vi "AT1B_Naeherung.vi"() -> ()   [LabVIEW 2026]
doc: "Virtueller Schlitten. NJ8 verwendet typische Daten, CJ8 und seitliche Geometrie sind einstellbare Beispiele. Erst Sensor und Probe waehlen, dann axial oder seitlich\nfahren. Nullsetzen aendert nur den Massstab."
panel:
  out "Bewegungsparameter gueltig":bool=TRUE
  out "Grafikfehlercode":i32
  out "Ausgangsspannung [V] - 20 ms je Punkt":dbl(graph)
  out "CSV-Fehlercode":i32
  out "Ungespeicherte Daten":bool
  out "Zeilen aufgenommen":i32
  out "Aufnahmestatus":string
  in  "Pruefstand beenden":bool
  in  "Neue CSV-Datei":path
  in  "CSV speichern":bool
  in  "Ungespeicherte Aufnahme verwerfen erlauben":bool
  in  "Neue Aufnahme":bool
  in  "Aufnahme eingeschaltet":bool
  out "Signalzustand":string="Mit Ausfuehren / Strg+R starten."
  out "Messung angehalten - Anzeige historisch":bool
  out "Massstab x [mm]":dbl=nan
  out "Massstab s [mm]":dbl=nan
  out "Ausgangsspannung [V]":dbl=nan
  out "Schaltausgang":bool
  in  "Messung eingeschaltet":bool=TRUE
  in  "Materialfaktor (-1 = Vorbelegung)":dbl=-1.0
  in  "Massstab x nullen":bool
  in  "Massstab s nullen":bool
  in  "Seitliche Reichweite [mm] - Beispiel":dbl=12.0
  in  "Hysterese-Anteil - Beispiel":dbl=0.075
  in  "CJ8 Empfindlichkeit [0..1]":dbl=0.5
  in  "Sensor eingeschaltet":bool=TRUE
  in  "Probenbreite [mm] (24 oder 40)":dbl=24.0
  in  "Andere Achse [mm]":dbl
  in  "Bewegte Achse":enum16{"Axial s", "Seitlich x"}(ring)
  in  "Probe (NJ8 / CJ8 Reihenfolge)":T1(ring)
  in  "Sensor":enum16{"NJ8 induktiv", "CJ8 kapazitiv"}(ring)
  out "Abgeschlossene Fahrten":dbl
  out "Fahrt aktiv":bool
  out "Position aktuell":dbl
  in  "Bewegung pausieren":bool
  in  "Bewegung stoppen":bool
  in  "Ablauf starten":bool
  in  "Schrittweite":dbl=0.1
  in  "Fahrtart":enum16{"Pendeln", "Schritte", "Einfachfahrt"}(ring)
  in  "Wiederholungen":dbl=1.0
  in  "Haltezeit [s]":dbl=0.5
  in  "Tempo pro Sekunde":dbl=1.0
  in  "Endposition":dbl
  in  "Startposition":dbl=20.0
  in  "Position setzen":bool
  in  "Handposition":dbl=20.0
  out "Kurzhilfe":string="Virtueller Schlitten. NJ8 verwendet typische Daten, CJ8 und seitliche Geometrie sind einstellbare Beispiele. Erst Sensor und Probe waehlen, dann axial oder seitlich\nfahren. Nullsetzen aendert nur den Massstab."
  out "Pruefstand":string="AT-1B / Induktiv und kapazitiv - Wegwerte in mm"
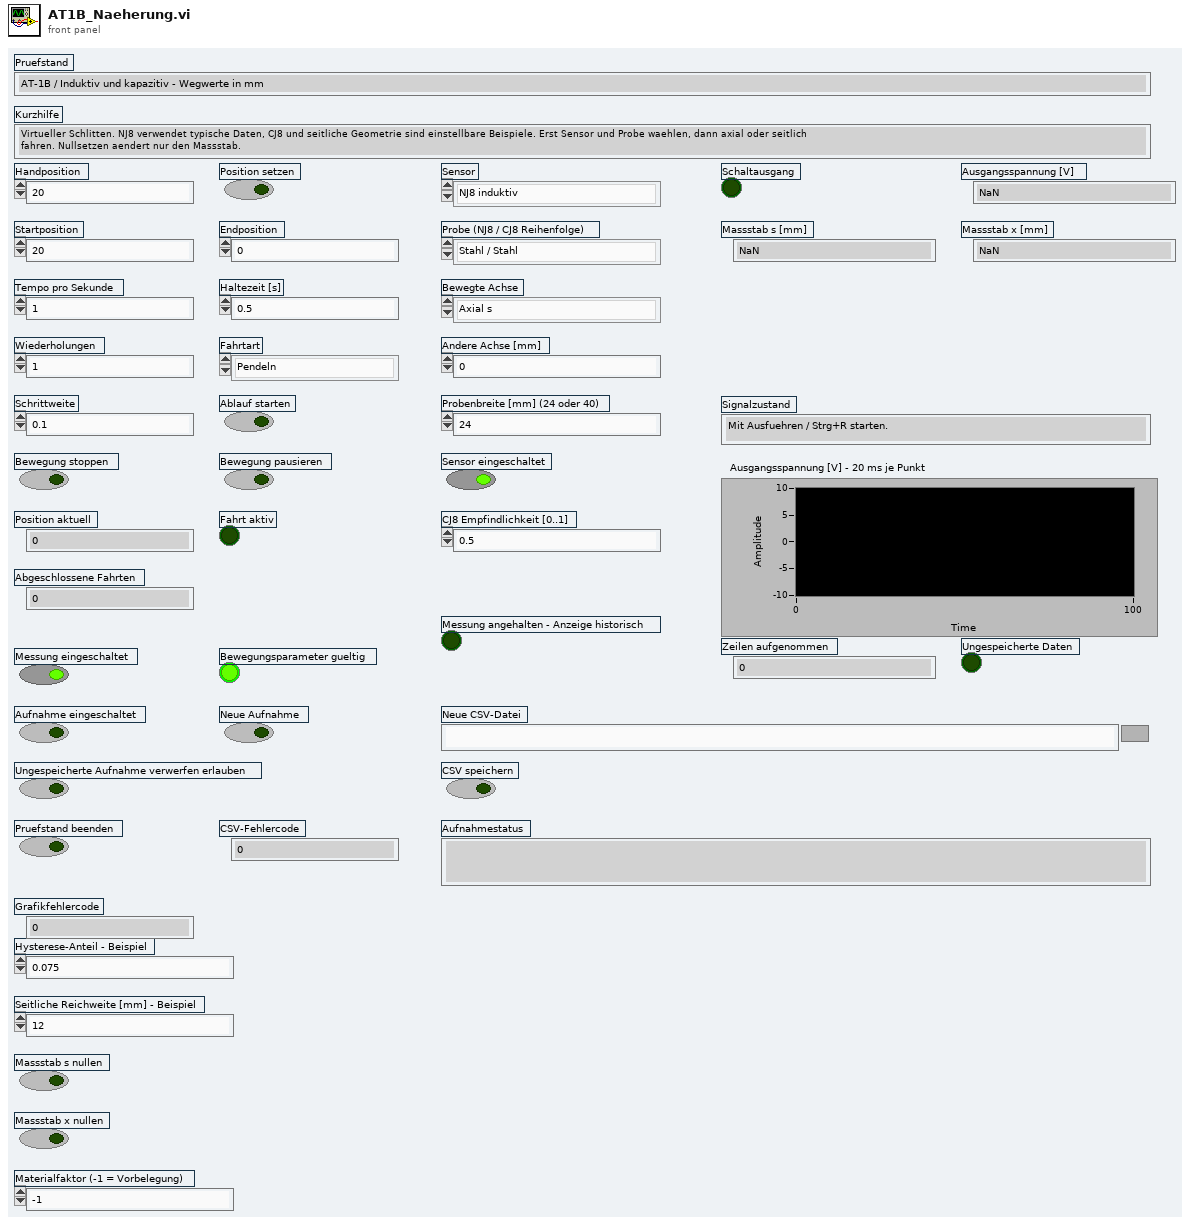
[diagram p1: front panel]
types:
  T1 = enum16{"Stahl / Stahl", "Kupfer / Weiss 6 mm", "Alu / Schwarz", "Magnet / Klar 8 mm", "Messing / Pappe", "V2A / V2A", "Magnet (nur CJ8)"}
  T2 = cluster{"record":bool, "clear":bool, "limit":i32, "header":string, "source":string}
diagram:
  n1 = while {
    shift-right: [w27] -> _
    shift-left: dbl[] [0.0, 0.0, 0.0, 0.0, 0.0, 0.0, 0.0, 0.0, 0.0, 0.0, 0.0, 0.0] -> [w26]
    shift-right: [w83] -> _
    shift-left: dbl[] [0.0, 0.0, 0.0, 0.0, 0.0] -> [w82]
    shift-right: [w88] -> _
    shift-left: dbl[] [nan, nan, nan, nan] -> [w87]
    shift-right: [w128] -> _
    shift-left: cluster{"text":string, "count":i32} {"text"="Quelle;Zeit_s;Physisch_s_mm;Physisch_x_mm;Schaltausgang;Spannung_V;Massstab_s_mm;Massstab_x_mm;Qualitaet;Eingang_normal_s_mm;Eingang_lateral_x_mm;Eingang_specimen_width_mm;Eingang_material_index;Eingang_power;Eingang_supply_V;Eingang_sensitivity_0_to_1;Eingang_device_0_NJ8_1_CJ8;Eingang_hysteresis_fraction_example;Eingang_lateral_radius_mm_example;Eingang_zero_normal_pressed;Eingang_zero_lateral_pressed;Eingang_material_factor_override_negative_default\r\n", "count"=0} -> [w127]
    shift-right: [w130] -> _
    shift-left: 0 -> [w129]
    shift-right: [w177] -> _
    shift-left: errorcluster {"status"=FALSE, "code"=0, "source"=""} -> [w176]
    i -> [w7]
    stop <- w193 stop-if-true
    w10 = FALSE
    (unwired) 1.0
    w9 = 0.0
    # "Virtueller Pruefstand - 20 ms Modellschritt"
    n2 = case shown="True" "Position setzen" {
      frame False {
      }
      frame True {
        n3 = property on="Position setzen" class="Bool. (strikt)"("Value"=FALSE) -> ()  [unwired: 2 in, 2 out]
      }
    }
    n4 = case shown="True" "Ablauf starten" {
      frame False {
      }
      frame True {
        n5 = property on="Ablauf starten" class="Bool. (strikt)"("Value"=FALSE) -> ()  [unwired: 2 in, 2 out]
      }
    }
    n6 = case shown="True" "Bewegung stoppen" {
      frame False {
      }
      frame True {
        n7 = property on="Bewegung stoppen" class="Bool. (strikt)"("Value"=FALSE) -> ()  [unwired: 2 in, 2 out]
      }
    }
    n8 = case shown="True" "Massstab s nullen" {
      frame False {
      }
      frame True {
        n9 = property on="Massstab s nullen" class="Bool. (strikt)"("Value"=FALSE) -> ()  [unwired: 2 in, 2 out]
      }
    }
    n10 = case shown="True" "Massstab x nullen" {
      frame False {
      }
      frame True {
        n11 = property on="Massstab x nullen" class="Bool. (strikt)"("Value"=FALSE) -> ()  [unwired: 2 in, 2 out]
      }
    }
    n12 = case shown="True" "Neue Aufnahme" {
      frame False {
      }
      frame True {
        n13 = property on="Neue Aufnahme" class="Bool. (strikt)"("Value"=FALSE) -> ()  [unwired: 2 in, 2 out]
      }
    }
    n14 = case shown="True" "CSV speichern" {
      frame False {
      }
      frame True {
        n15 = property on="CSV speichern" class="Bool. (strikt)"("Value"=FALSE) -> ()  [unwired: 2 in, 2 out]
      }
    }
    n16 = case shown="True" "Pruefstand beenden" {
      frame False {
      }
      frame True {
        n17 = property on="Pruefstand beenden" class="Bool. (strikt)"("Value"=FALSE) -> ()  [unwired: 2 in, 2 out]
      }
    }
    n18 = Wait (ms)(milliseconds to wait=u32 20) -> ()  [unwired: 1 out]
    n19 = Select(t=1.0, s="Ablauf starten", f=0.0) -> (s? t:f=w30:dbl)
    n20 = property on="Ausgangsspannung [V] - 20 ms je Punkt" class="SVDiagr (strikt)"("Legend:Visible"=w10, "Palette:Visible"=w10, "Scale Legend:Visible"=w10, "Position"=cluster{"Left":i32, "Top":i32} {"Left"=735, "Top"=420}, "Plot Area:Size"=cluster{"Width":u32, "Height":u32} {"Width"=340, "Height"=110}) -> (error out=w211:errorcluster)  [unwired: 2 in, 1 out]
    n21 = Select(t=1.0, s="Bewegung pausieren", f=0.0) -> (s? t:f=w33:dbl)
    n22 = Select(t=1.0, s="Position setzen", f=0.0) -> (s? t:f=w36:dbl)
    n23 = Select(t=1.0, s="Bewegung stoppen", f=0.0) -> (s? t:f=w39:dbl)
    n24 = Greater?(x="Bewegte Achse", y=0.0) -> (0:w69:bool)
    n25 = Select(t=1.0, s="Sensor eingeschaltet", f=0.0) -> (s? t:f=w74:dbl)
    n26 = Select(t=1.0, s="Massstab s nullen", f=0.0) -> (s? t:f=w78:dbl)
    n27 = Select(t=1.0, s="Massstab x nullen", f=0.0) -> (s? t:f=w81:dbl)
    n28 = Not(x="Messung eingeschaltet") -> (.not. x?=→"Messung angehalten - Anzeige historisch":bool)
    n29 = And(x="Aufnahme eingeschaltet", y="Messung eingeschaltet") -> (x .and. y?=w139:bool)
    n30 = Unbundle By Name(w127) -> ("count"=w131:i32)  [unwired: 1 out]
    n31 = Equal?(x=w7, y=w9) -> ()  [unwired: 1 out]
    n32 = Quotient & Remainder(x=w7, y=5) -> (x-y*floor(x/y)=w137:i32)  [unwired: 1 out]
    n33 = Build Array(0.02, "Startposition", "Endposition", "Tempo pro Sekunde", "Haltezeit [s]", "Wiederholungen", w30, w33, w36, "Handposition", "Fahrtart", "Schrittweite", w39) -> (w40:dbl[])
    n34 = Unbundle By Name(w211) -> ("code"=→"Grafikfehlercode":i32)
    n35 = Greater?(x=w131, y=w129) -> (0:w132:bool)
    n36 = Equal?(x=w137, y=w9) -> (x = y?=w138:bool)
    n37 = call "Trajektorie.vi"("StateIn"=w26, "Parameters"=w40) -> ("Values"=w41:dbl[], "StateOut"=w27:dbl[])  [unwired: 8 in]
    n38 = Not(x=w132) -> (.not. x?=w133:bool)
    n39 = And(x=w139, y=w138) -> (x .and. y?=w140:bool)
    n40 = Index Array(array=w41, index=0) -> (element=w43:dbl)
    "Position aktuell" <- w43
    n41 = Index Array(array=w41, index=3) -> (element=w45:dbl)
    n42 = Index Array(array=w41, index=4) -> (element=w47:dbl)
    n43 = Index Array(array=w41, index=1) -> (element=w51:dbl)
    n44 = Index Array(array=w41, index=2) -> (element=→"Abgeschlossene Fahrten":dbl)
    n45 = Or(x=w133, y="Ungespeicherte Aufnahme verwerfen erlauben") -> (x .or. y?=w134:bool)
    n46 = Greater?(x=w47, y=0.0) -> (0:→"Bewegungsparameter gueltig":bool)
    n47 = Greater?(x=w51, y=0.0) -> (0:→"Fahrt aktiv":bool)
    n48 = Select(t="Andere Achse [mm]", s=w69, f=w43) -> (s? t:f=w70:dbl)
    n49 = Select(t=w43, s=w69, f="Andere Achse [mm]") -> (s? t:f=w71:dbl)
    n50 = And(x="Neue Aufnahme", y=w134) -> (x .and. y?=w135:bool)
    n51 = Not(x=w134) -> (.not. x?=w194:bool)
    n52 = Build Array(w70, w71, "Probenbreite [mm] (24 oder 40)", "Probe (NJ8 / CJ8 Reihenfolge)", w74, 24.0, "CJ8 Empfindlichkeit [0..1]", "Sensor", "Hysterese-Anteil - Beispiel", "Seitliche Reichweite [mm] - Beispiel", w78, w81, "Materialfaktor (-1 = Vorbelegung)") -> (w84:dbl[])
    n53 = Bundle By Name(cluster=T2 {"record"=FALSE, "clear"=FALSE, "limit"=10000, "header"="", "source"=""}, "record"=w140, "clear"=w135, "limit"=10000, "header"="Quelle;Zeit_s;Physisch_s_mm;Physisch_x_mm;Schaltausgang;Spannung_V;Massstab_s_mm;Massstab_x_mm;Qualitaet;Eingang_normal_s_mm;Eingang_lateral_x_mm;Eingang_specimen_width_mm;Eingang_material_index;Eingang_power;Eingang_supply_V;Eingang_sensitivity_0_to_1;Eingang_device_0_NJ8_1_CJ8;Eingang_hysteresis_fraction_example;Eingang_lateral_radius_mm_example;Eingang_zero_normal_pressed;Eingang_zero_lateral_pressed;Eingang_material_factor_override_negative_default\r\n", "source"="AT1B_Naeherung;") -> (w145:T2)
    n54 = Select(t=errorcluster {"status"=FALSE, "code"=0, "source"=""}, s=w135, f=w176) -> (s? t:f=w182:errorcluster)
    n55 = Select(t=0, s=w135, f=w129) -> (s? t:f=w189:i32)
    n56 = And(x="Neue Aufnahme", y=w194) -> (x .and. y?=w195:bool)
    n57 = call "Naeherung_Schritt.vi"("StateIn"=w82, "Parameters"=w84) -> ("Values"=w85:dbl[], "StateOut"=w83:dbl[])  [unwired: 8 in]
    n58 = Index Array(array=w84, index=0) -> (element=w147:dbl)
    n59 = Index Array(array=w84, index=1) -> (element=w149:dbl)
    n60 = Index Array(array=w84, index=2) -> (element=w151:dbl)
    n61 = Index Array(array=w84, index=3) -> (element=w153:dbl)
    n62 = Index Array(array=w84, index=4) -> (element=w155:dbl)
    n63 = Index Array(array=w84, index=5) -> (element=w157:dbl)
    n64 = Index Array(array=w84, index=6) -> (element=w159:dbl)
    n65 = Index Array(array=w84, index=7) -> (element=w161:dbl)
    n66 = Index Array(array=w84, index=8) -> (element=w163:dbl)
    n67 = Index Array(array=w84, index=9) -> (element=w165:dbl)
    n68 = Index Array(array=w84, index=10) -> (element=w167:dbl)
    n69 = Index Array(array=w84, index=11) -> (element=w169:dbl)
    n70 = Index Array(array=w84, index=12) -> (element=w171:dbl)
    n71 = Select(t=w85, s="Messung eingeschaltet", f=w87) -> (s? t:f=w88:dbl[])
    n72 = Index Array(array=w85, index=0) -> (element=w90:dbl)
    n73 = Index Array(array=w85, index=4) -> (element=w101:dbl)
    n74 = Index Array(array=w85, index=0) -> (element=w112:dbl)
    n75 = Index Array(array=w85, index=1) -> (element=w114:dbl)
    n76 = Index Array(array=w85, index=2) -> (element=w116:dbl)
    n77 = Index Array(array=w85, index=3) -> (element=w118:dbl)
    n78 = Index Array(array=w85, index=4) -> (element=w120:dbl)
    n79 = Greater?(x=w90, y=0.0) -> (0:→"Schaltausgang":bool)
    n80 = Index Array(array=w88, index=1) -> (element=→"Ausgangsspannung [V]":dbl)
    n81 = Index Array(array=w88, index=2) -> (element=→"Massstab s [mm]":dbl)
    n82 = Index Array(array=w88, index=3) -> (element=→"Massstab x [mm]":dbl)
    n83 = Equal?(x=w101, y=1.0) -> (x = y?=w104:bool)
    n84 = Equal?(x=w101, y=2.0) -> (x = y?=w108:bool)
    n85 = Build Array(w45, w70, w71, w112, w114, w116, w118, w120, w147, w149, w151, w153, w155, w157, w159, w161, w163, w165, w167, w169, w171) -> (w172:dbl[])
    n86 = Index Array(array=w88, index=1) -> (element=→"Ausgangsspannung [V] - 20 ms je Punkt":dbl)
    n87 = Select(t="Messsignal gueltig - Beispielkennlinie", s=w104, f="Parameter ungueltig - Eingaben pruefen.") -> (s? t:f=w106:string)
    n88 = call "Aufzeichnung_Schritt.vi"("Previous"=w127, "Row"=w172, "Settings"=w145) -> ("Full"=w173:bool, "Current"=w128:cluster{"text":string, "count":i32})  [unwired: 11 in]
    n89 = Select(t="Sensor ausgeschaltet", s=w108, f=w106) -> (s? t:f=→"Signalzustand":string)
    n90 = Unbundle By Name(w128) -> ("text"=w174:string, "count"=w175:i32)
    "Zeilen aufgenommen" <- w175
    n91 = Greater?(x=w175, y=0.0) -> (0:w179:bool)
    n92 = And(x="CSV speichern", y=w179) -> (x .and. y?=w180:bool)
    n93 = case shown="True" w180 {
      tunnel: "Neue CSV-Datei" -> [_ w214]
      tunnel: w182 -> [w213 _]
      tunnel: w174 -> [_ w215]
      tunnel: [w213 w216] -> w177
      frame False {
      }
      frame True {
        n94 = call "CSV_Speichern.vi"("Text"=w215, "Datei"=w214) -> ("error out"=w216:errorcluster)  [unwired: 13 in]
      }
    }
    n95 = Unbundle By Name(w177) -> ("status"=w183:bool, "code"=→"CSV-Fehlercode":i32, "source"=w185:string)
    n96 = Not(x=w183) -> (.not. x?=w186:bool)
    n97 = And(x=w180, y=w186) -> (x .and. y?=w187:bool)
    n98 = Select(t=w175, s=w187, f=w189) -> (s? t:f=w130:i32)
    n99 = Greater?(x=w175, y=w130) -> (0:w190:bool)
    "Ungespeicherte Daten" <- w190
    n100 = Not(x=w190) -> (.not. x?=w191:bool)
    n101 = Select(t="Aufnahme noch nicht gespeichert. Vor neuer Aufnahme oder Beenden CSV speichern oder Verwerfen erlauben einschalten.", s=w190, f="Bereit. Aufnahme mit neuem Dateinamen speichern.") -> (s? t:f=w201:string)
    n102 = Or(x=w191, y="Ungespeicherte Aufnahme verwerfen erlauben") -> (x .or. y?=w192:bool)
    n103 = Select(t="Aufnahme voll (10 000 Zeilen). Speichern und neue Aufnahme beginnen.", s=w173, f=w201) -> (s? t:f=w203:string)
    n104 = And(x="Pruefstand beenden", y=w192) -> (x .and. y?=w193:bool)
    n105 = Not(x=w193) -> (.not. x?=w196:bool)
    n106 = And(x="Pruefstand beenden", y=w196) -> (x .and. y?=w197:bool)
    n107 = Or(x=w195, y=w197) -> (x .or. y?=w198:bool)
    n108 = Select(t="Erst CSV speichern oder Verwerfen erlauben einschalten.", s=w198, f=w203) -> (s? t:f=w205:string)
    n109 = Select(t=w185, s=w183, f=w205) -> (s? t:f=→"Aufnahmestatus":string)
    "Pruefstand" <- "AT-1B / Induktiv und kapazitiv - Wegwerte in mm"
    "Kurzhilfe" <- "Virtueller Schlitten. NJ8 verwendet typische Daten, CJ8 und seitliche Geometrie sind einstellbare Beispiele. Erst Sensor und Probe waehlen, dann axial oder seitlich\nfahren. Nullsetzen aendert nur den Massstab."
  }
